vi "Untitled 1.vi"() -> ()   [LabVIEW 2023]
panel:
  out "Application Directory":path
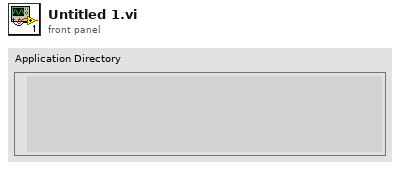
[diagram p1: front panel]
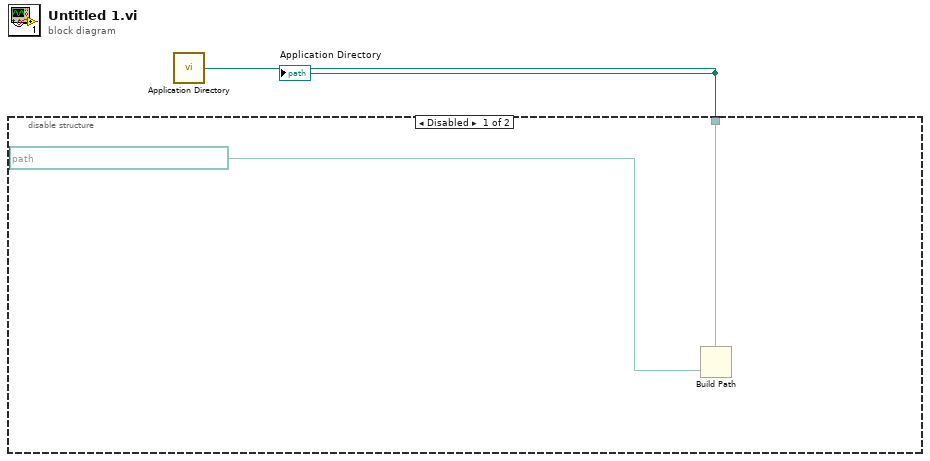
[diagram p0: block diagram]
diagram:
  n1 = call <vilib>:"Application Directory.vi"() -> ("Application Directory"=w1:path)
  "Application Directory" <- w1
  n2 = disable-structure shown="Disabled" {
    disable-tunnel: w1 -> [w2 _]
    frame Disabled {
      n3 = Build Path(base path=w2, name or relative path=path "hp8903b 生成xy图像（低频）.vi") -> ()  [unwired: 1 out]
    }
    frame Enabled {
    }
  }
